vi "Init.vi"(8 "error in (no error)":errorcluster, 11 "config":T2={"connection"={"host"="", "channel"=2, "cert path"=path "/home/lvuser/cansub_root_cert.crt"}, "bit rates"={"nominal bit rate"=500000, "nominal sample point"=80.0, "data bit rate"=2000000, "data sample point"=80.0}, "listen only"=FALSE, "filters"=[], "read mode"=enum."Poll", "max bytes per read"=4096, "reader FIFO depth"=0, "reader priority"=0, "ownership"=enum."Direct"} {"filters"."f2" format="%.0x"; "filters"."f1" format="%.0x"}) -> (0 "error out":errorcluster, 2 "bit timing":T1, 3 "channel out":refnum<class "CANsub_Channel.lvclass">)   [LabVIEW 2021, in "CANsub_API.lvlib" / "CANsub_Channel.lvclass"]
doc: "Makes a CANsub channel object from a config. Checks the config (5207 for features not built yet: listen only, filter lists, Reader mode, Shared ownership), computes the bit timing (W9). Returns a CANsub_DirectChannel on a CANsub_Channel wire. No I/O. Setup/teardown only: do not call in a periodic loop (allocates, may block)."
uses:
  CANsub_Channel.lvclass
  CANsub_DirectChannel/CANsub_DirectChannel.lvclass
  C:/Dev/CIF/CAN_RW_CANsub/src/CANsub/c_client/api/CANsub_Channel/CANsub_Channel.lvclass
  CANsub_C.lvlib
  Typedefs/CANsub_Read_Mode.ctl
  CANsub_API.lvlib
  Typedefs/CANsub_Ownership.ctl
  common/Typedefs/CANsub_connection.ctl
  common/CANsub_Common.lvlib
  common/Typedefs/CANsub_Bit_Rates.ctl
  Typedefs/CANsub_Filter.ctl
  Typedefs/CANsub_Config.ctl
  common/Typedefs/Bit_Timing.ctl
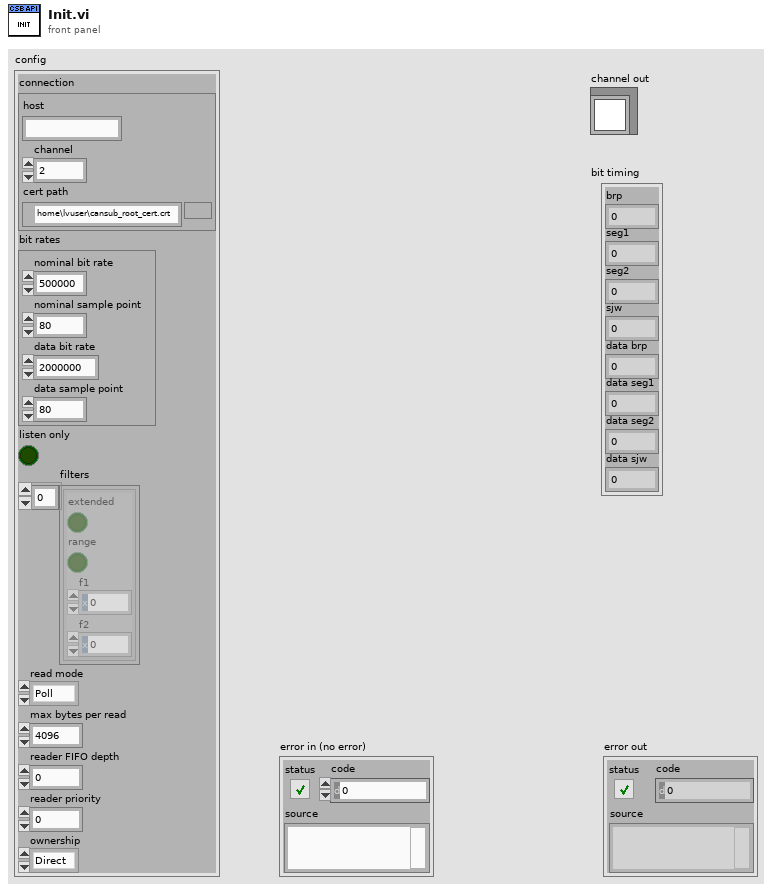
[diagram p1: front panel]
types:
  T1 = typedef "CANsub_Common.lvlib/Bit_Timing.ctl" = cluster{"brp":u16, "seg1":u16, "seg2":u16, "sjw":u16, "data brp":u16, "data seg1":u16, "data seg2":u16, "data sjw":u16}
  T2 = typedef "CANsub_API.lvlib/CANsub_Config.ctl" = cluster{"connection":T3, "bit rates":T4, "listen only":bool, "filters":T5[], "read mode":T6, "max bytes per read":i32, "reader FIFO depth":i32, "reader priority":i32, "ownership":T7}
  T3 = typedef "CANsub_Common.lvlib/CANsub_connection.ctl" = cluster{"host":string, "channel":u8, "cert path":path}
  T4 = typedef "CANsub_Common.lvlib/CANsub_Bit_Rates.ctl" = cluster{"nominal bit rate":u32, "nominal sample point":dbl, "data bit rate":u32, "data sample point":dbl}
  T5 = typedef "CANsub_API.lvlib/CANsub_Filter.ctl" = cluster{"extended":bool, "range":bool, "f1":u32, "f2":u32}
  T6 = typedef "CANsub_API.lvlib/CANsub_Read_Mode.ctl" = enum16{"Poll", "Reader"}
  T7 = typedef "CANsub_API.lvlib/CANsub_Ownership.ctl" = enum16{"Direct", "Shared"}
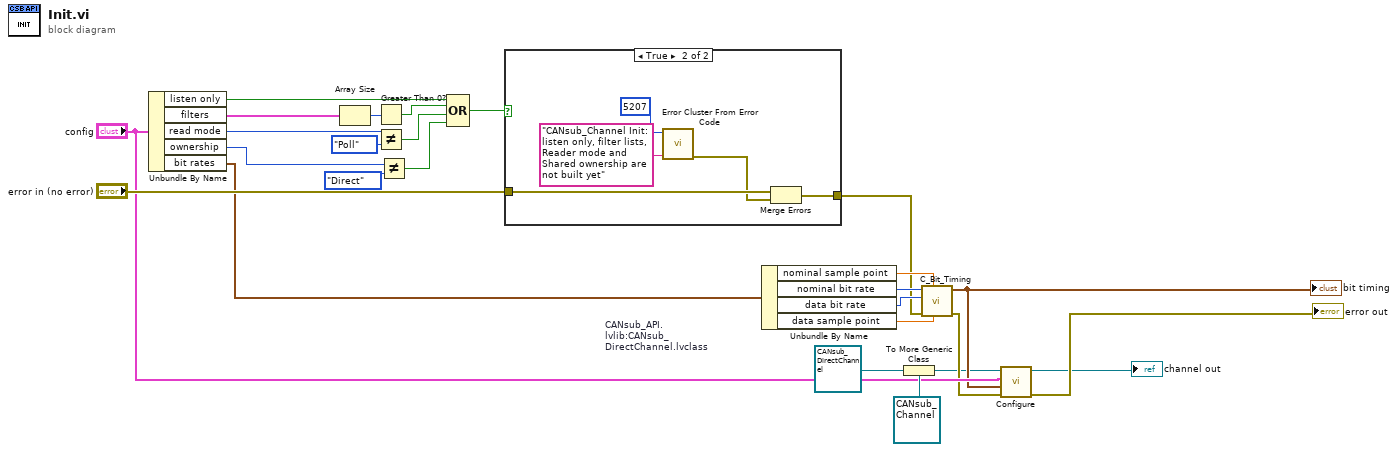
[diagram p0: block diagram]
diagram:
  w3 = refnum<class "CANsub_DirectChannel.lvclass"> refnum  # CANsub_API.lvlib:CANsub_DirectChannel.lvclass
  n1 = Unbundle By Name("config") -> ("listen only"=w20:bool, "filters"=w26:T5[], "read mode"=w24:T6, "ownership"=w22:T7, "bit rates"=w14:T4)
  n2 = Array Size(array=w26) -> (size(s)=w25:i32)
  n3 = Greater Than 0?(x=w25) -> (x > 0?=w19:bool)
  n4 = Not Equal?(x=w24, y=CANsub_Read_Mode."Poll" ("read mode")) -> (x != y?=w18:bool)
  n5 = Not Equal?(x=w22, y=CANsub_Ownership."Direct") -> (x != y?=w17:bool)
  n6 = Compound Arithmetic op=OR(w20, w19, w18, w17) -> (w16:bool)
  n7 = case shown="True" w16 {
    tunnel: "error in (no error)" -> [w27 w30]
    tunnel: [w27 w28] -> w9
    frame False {
    }
    frame True {
      n8 = call <vilib>:"Error Cluster From Error Code.vi"("error message (\"\")"="CANsub_Channel Init: listen only, filter lists, Reader mode and Shared ownership are not built yet" ("error message (\"\")"), "error code (0)"=5207) -> ("error out"=w29:errorcluster)  [unwired: 7 in]
      n9 = Merge Errors(w30, w29) -> (w28:errorcluster)
    }
  }
  n10 = Unbundle By Name(w14) -> ("nominal sample point"=w13:dbl, "nominal bit rate"=w12:u32, "data bit rate"=w11:u32, "data sample point"=w10:dbl)
  n11 = To More Generic Class(target class=refnum<class "CANsub_Channel.lvclass"> refnum ("CANsub_API.lvlib:CANsub_Channel.lvclass"), reference=w3) -> (generic class reference=w2:refnum<class "CANsub_Channel.lvclass">)
  n12 = call "C_Bit_Timing.vi"("data sample point"=w10, "nominal sample point"=w13, "error in (no error)"=w9, "data bit rate"=w11, "nominal bit rate"=w12) -> ("error out"=w5:errorcluster, "Bit_Timing"=w6:T1)  [unwired: 3 in, 2 out]
  "bit timing" <- w6
  n13 = call-dynamic "Configure.vi"("error in (no error)"=w5, "bit timing"=w6, "config"="config", "channel in"=w2) -> ("error out"=→"error out":errorcluster, "channel out"=→"channel out":refnum<class "CANsub_Channel.lvclass">)  [unwired: 6 in]
